vi "Test Play Wav.vi"() -> ()   [LabVIEW 2019]
uses:
  Libraries/LibSDL2 Wrapper/LibSDL2.lvlib
  Libraries/LibSDL2 Wrapper/Controls/Init Flags.ctl
  Libraries/LibSDL2_Mixer Wrapper/LibSDL2_Mixer.lvlib
panel:
  out "Return":i32
  out "Chunk Pointer":u32 format="%.0x"
  out "Error":string
  out "Flags Successfully Initialised":i32 format="%.0x"
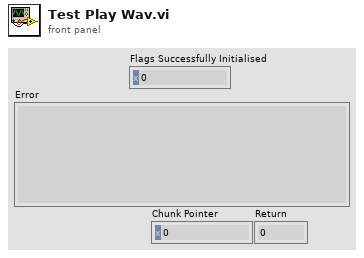
[diagram p1: front panel]
types:
  T1 = typedef "LibSDL2.lvlib/Init Flags.ctl" = u32
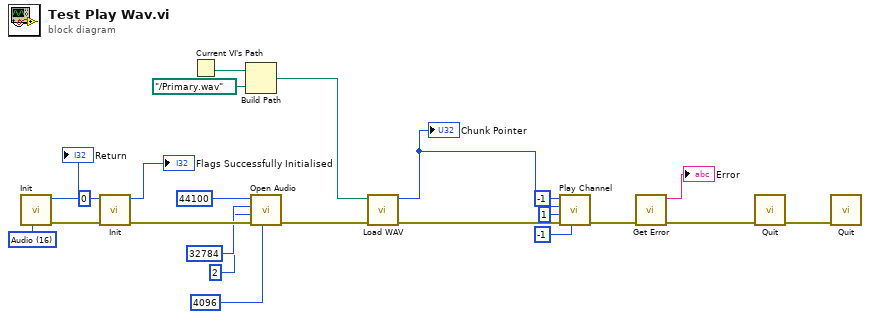
[diagram p0: block diagram]
diagram:
  w23 = T1 16 items=["Timer"=1, "Audio"=16, "Video"=32, "Joystick"=512, "Haptic"=4096, "Game Controller"=8192, "Events"=16384, "No Parachute"=1048576, "Everything"=17244689] ("Init Flags")
  n1 = call "Init.vi"("Flags"=w23) -> ("error out"=w22:errorcluster, "Return"=→"Return":i32)  [unwired: 9 in]
  n2 = call "Init.vi"("error in"=w22, "Flags"=0) -> ("error out"=w13:errorcluster, "Flags Successfully Initialised"=→"Flags Successfully Initialised":i32)  [unwired: 8 in]
  n3 = Current VI's Path() -> (path=w18:path)
  n4 = Build Path(base path=w18, name or relative path=path "../Primary.wav") -> (appended path=w16:path)
  n5 = call "Open Audio.vi"("Chunksize"=4096, "error in"=w13, "Channels"=2, "Format"=u16 32784, "Frequency"=44100) -> ("error out"=w12:errorcluster)  [unwired: 5 in, 1 out]
  n6 = call "Load WAV.vi"("error in"=w12, "File"=w16) -> ("error out"=w3:errorcluster, "Chunk Pointer"=w7:u32)  [unwired: 8 in]
  "Chunk Pointer" <- w7
  n7 = call "Play Channel.vi"("Ticks"=-1, "error in"=w3, "Loops"=1, "Chunk Pointer"=w7, "Channel"=-1) -> ("error out"=w2:errorcluster)  [unwired: 5 in, 1 out]
  n8 = call "Get Error.vi"("error in"=w2) -> ("error out"=w1:errorcluster, "Error"=→"Error":string)  [unwired: 9 in]
  n9 = call "Quit.vi"("error in"=w1) -> ("error out"=w14:errorcluster)  [unwired: 10 in]
  n10 = call "Quit.vi"("error in"=w14) -> ()  [unwired: 10 in, 1 out]
